vi "Periodic Tasks.vi"(8 "error in (no error)":errorcluster) -> ()   [LabVIEW 2016]
doc: "This VI runs in parallel to other tasks. It can contain as many user-defined periodic loops as you need. These can carry out PID or other sorts of timed response."
uses:
  Extra/TypeDefs/GatePos_Type.ctl
  Extra/TypeDefs/RobotParameters.ctl
  Extra/TypeDefs/GateParameters_Type.ctl
  ArgosLib/Miscellaneous/TypeDefs/MotorLimitPositions_Type.ctl
  Extra/TypeDefs/RailParameters_Type.ctl
  ArgosLib/Sensors/Ultrasonic/TypeDefs/UltrasonicParameters_Type.ctl
  Extra/TypeDefs/DB/dbParams_Type.ctl
  Extra/TypeDefs/AutoMode_Type.ctl
  ArgosLib/Drive/MotorControl/TypeDefs/RobotDriveMotorSelectorEnum.ctl
  Extra/TypeDefs/GearCollectState_Type.ctl
  Extra/TypeDefs/DB/dbButtonDisplayNames_Type.ctl
  Extra/TypeDefs/DB/dbStringDisplayNames_Type.ctl
  <vilib>/Rock Robotics/WPI/DriverStation/WPI_DriverStationRobotMode2.ctl
  Extra/TypeDefs/DB/dbSliderDisplayNames_Type.ctl
  <vilib>/Rock Robotics/WPI/ThirdParty/CanMotor/TalonSRX/WPI_CANTalonSRX_BrakeOverride.ctl
  Extra/Global_Var-RefNum/Global_Var_Drive.vi
  <vilib>/Rock Robotics/Network Tables/NT Write String.vi
  <vilib>/Rock Robotics/Network Tables/NT Read Boolean.vi
  <vilib>/Rock Robotics/Network Tables/NT Write Number.vi
  <vilib>/Rock Robotics/Network Tables/NT Write Boolean.vi
  Extra/Global_Var-RefNum/Global_Var_Other.vi
  <vilib>/Rock Robotics/Network Tables/NT Read String.vi
  Extra/Global_Var-RefNum/GlobalVar_LED.vi
  <vilib>/Rock Robotics/Network Tables/NT Read Number.vi
  ArgosLib/Miscellaneous/Arbitor/ArbitorSpecializations/Arbitor_Int.vi
  ArgosLib/Miscellaneous/Arbitor/ArbitorSpecializations/Arbitor_Float.vi
  ArgosLib/Miscellaneous/Arbitor/ArbitorSpecializations/Arbitor_Bool.vi
  ArgosLib/ArgosLib.lvlib
  Extra/Sensors/ADI MXP IMU/ADIS16448_IMU.lvlib
  Extra/Sensors/PixyCam/PixyCam_LabVIEW.lvlib
panel:
  in  "Continue_Forward_Distance":dbl=-15.0
  in  "BrakeMode?":bool
  in  "Turning_Angle":dbl=30.0
  in  "AutoMode":T1=enum."GearMiddle"
  in  "Reverse_Drive_Distance":dbl=-50.0 format="%#_13g"
  in  "Reverse_Drive_Speed":dbl=0.6 format="%#_13g"
  in  "Start_Auto?":bool
  in  "Robot Parameters":enum32{"Competition", "Practice"}(tab)
  in  "CompetitionRobotParameters":T2={"GateParameters"={"Scale Positions"={"Forward_StartScale"=1575.0, "Reverse_StartScale"=1440.0, "Forward_Limit"=1575.0, "Reverse_Limit"=1440.0}, "Catch_Pos"=1500.0, "Clamp_Pos"=1445.0, "Open_Pos"=1669.0, "Timeout (ms)"=750, "Invert?"=TRUE, "Scale_Factor"=0.01, "Acceptable_Range"=5.0}, "Rail Parameters"={"Scale Positions"={"Forward_StartScale"=15.4, "Reverse_StartScale"=8.7, "Forward_Limit"=21.4, "Reverse_Limit"=2.7}, "Motor_Limit"=0.6, "Invert?"=FALSE, "PID gains"={"proportional gain (Kc)"=0.2, "integral time (Ti, min)"=0.0, "derivative time (Td, min)"=0.0}, "Timeout (ms)"=2000, "CatchPosition"=6.5}, "Invert_Intake"=TRUE, "UltrasonicParameters"={"MedianFilterSamples"=8, "LowPassFilterPercent"=0.5, "RailOffset (in)"=4.0, "MaxRange (in)"=24.7}, "Feeder_Invert"=FALSE, "Drive PID Gains"={"proportional gain (Kc)"=0.04, "integral time (Ti, min)"=0.025, "derivative time (Td, min)"=1e-05}, "DriveSpeed_Invert"=TRUE, "DriveEncoder_Invert"=FALSE, "DefaultDBParams"={"MiddleAutoDist (in)"=-60.0, "SideAutoDist (in)"=-45.0, "AutoSpeed"=0.6, "RailCenterOffset (in)"=0.0, "RedAllianceRPM"=3550.0, "BlueAllianceRPM"=3400.0, "BaselineRPM"=3000.0}} {"Rail Parameters"."PID gains"."derivative time (Td, min)" format="%.3f"; "Rail Parameters"."PID gains"."integral time (Ti, min)" format="%.3f"; "Rail Parameters"."PID gains"."proportional gain (Kc)" format="%.3f"}
  in  "PracticeRobotParameters":T2={"GateParameters"={"Scale Positions"={"Forward_StartScale"=1700.0, "Reverse_StartScale"=1560.0, "Forward_Limit"=1700.0, "Reverse_Limit"=1560.0}, "Catch_Pos"=1620.0, "Clamp_Pos"=1585.0, "Open_Pos"=1680.0, "Timeout (ms)"=750, "Invert?"=TRUE, "Scale_Factor"=0.012, "Acceptable_Range"=5.0}, "Rail Parameters"={"Scale Positions"={"Forward_StartScale"=17.25, "Reverse_StartScale"=12.35, "Forward_Limit"=23.25, "Reverse_Limit"=6.35}, "Motor_Limit"=0.6, "Invert?"=FALSE, "PID gains"={"proportional gain (Kc)"=0.2, "integral time (Ti, min)"=0.0, "derivative time (Td, min)"=0.0}, "Timeout (ms)"=2000, "CatchPosition"=6.5}, "Invert_Intake"=FALSE, "UltrasonicParameters"={"MedianFilterSamples"=8, "LowPassFilterPercent"=0.5, "RailOffset (in)"=4.0, "MaxRange (in)"=27.0}, "Feeder_Invert"=FALSE, "Drive PID Gains"={"proportional gain (Kc)"=0.04, "integral time (Ti, min)"=0.025, "derivative time (Td, min)"=1e-05}, "DriveSpeed_Invert"=FALSE, "DriveEncoder_Invert"=TRUE, "DefaultDBParams"={"MiddleAutoDist (in)"=-60.0, "SideAutoDist (in)"=-45.0, "AutoSpeed"=0.6, "RailCenterOffset (in)"=0.0, "RedAllianceRPM"=3550.0, "BlueAllianceRPM"=3400.0, "BaselineRPM"=3000.0}} {"Rail Parameters"."PID gains"."derivative time (Td, min)" format="%.3f"; "Rail Parameters"."PID gains"."integral time (Ti, min)" format="%.3f"; "Rail Parameters"."PID gains"."proportional gain (Kc)" format="%.3f"}
  out "Ultrasonic":T8(graph)={"UltrasonicRange (in)"=1.824963579811325, "MedianOnly_UltrasonicRange (in)"=1.4520408163265301, "Unfiltered_UltrasonicRange (in)"=1.4513605442176853}
  in  "Manual_Track_Position":bool
  in  "Gear_Beam_Break_Sensor_Triggered":bool=TRUE
  in  "Reset_Encoder?":bool
  out "Dist_Travelled (In)":dbl
  out "Encoder Position":dbl
  out "Gear_Orientation_Bb_True?":bool
  in  "Manual_Gate_Control":T9
  out "Distance":dbl=-3.5761161830654182
  in  "GearRailWantedPosition":dbl(slide)=25.0 scale=5.0..25.0
  in  "ResetGearCollect":bool
  in  "ResetGearPlacer":bool
  in  "StartGearPlace":bool=TRUE
  in  "Place":bool=TRUE
  in  "Collect":bool=TRUE
  in  "Manual":bool
  in  "StartGearCollect":bool=TRUE
  out "GateReached":bool=TRUE
  out "IMU Angles Out":T10={"X Angle"=107.18836227857514, "Y Angle"=-158.5508446973779, "Z Angle"=83.6587271935076}
  # "Previous Values\nFwd_StartScale=1700\nReverse_StartScale=1560\nFwd_Limit=1700\nReverse_Limit=1560\nCatch=1604\nClamp=1570\nOpen=1669\nTimeout=750"
  # "1/24/17 (2014 Chassis)\nKc=0.015\nTi=5\nTd=0.0005\nTurns slowly, but well"
  # "2014 Chassis\nKc=0.09\nTi=0.9\nTd=0.001\nNot good for turning"
  # "2/12/17 (2017 Chassis)\nKc= 0.04\nTi=.025\nTd=1E-5\ndrives straight"
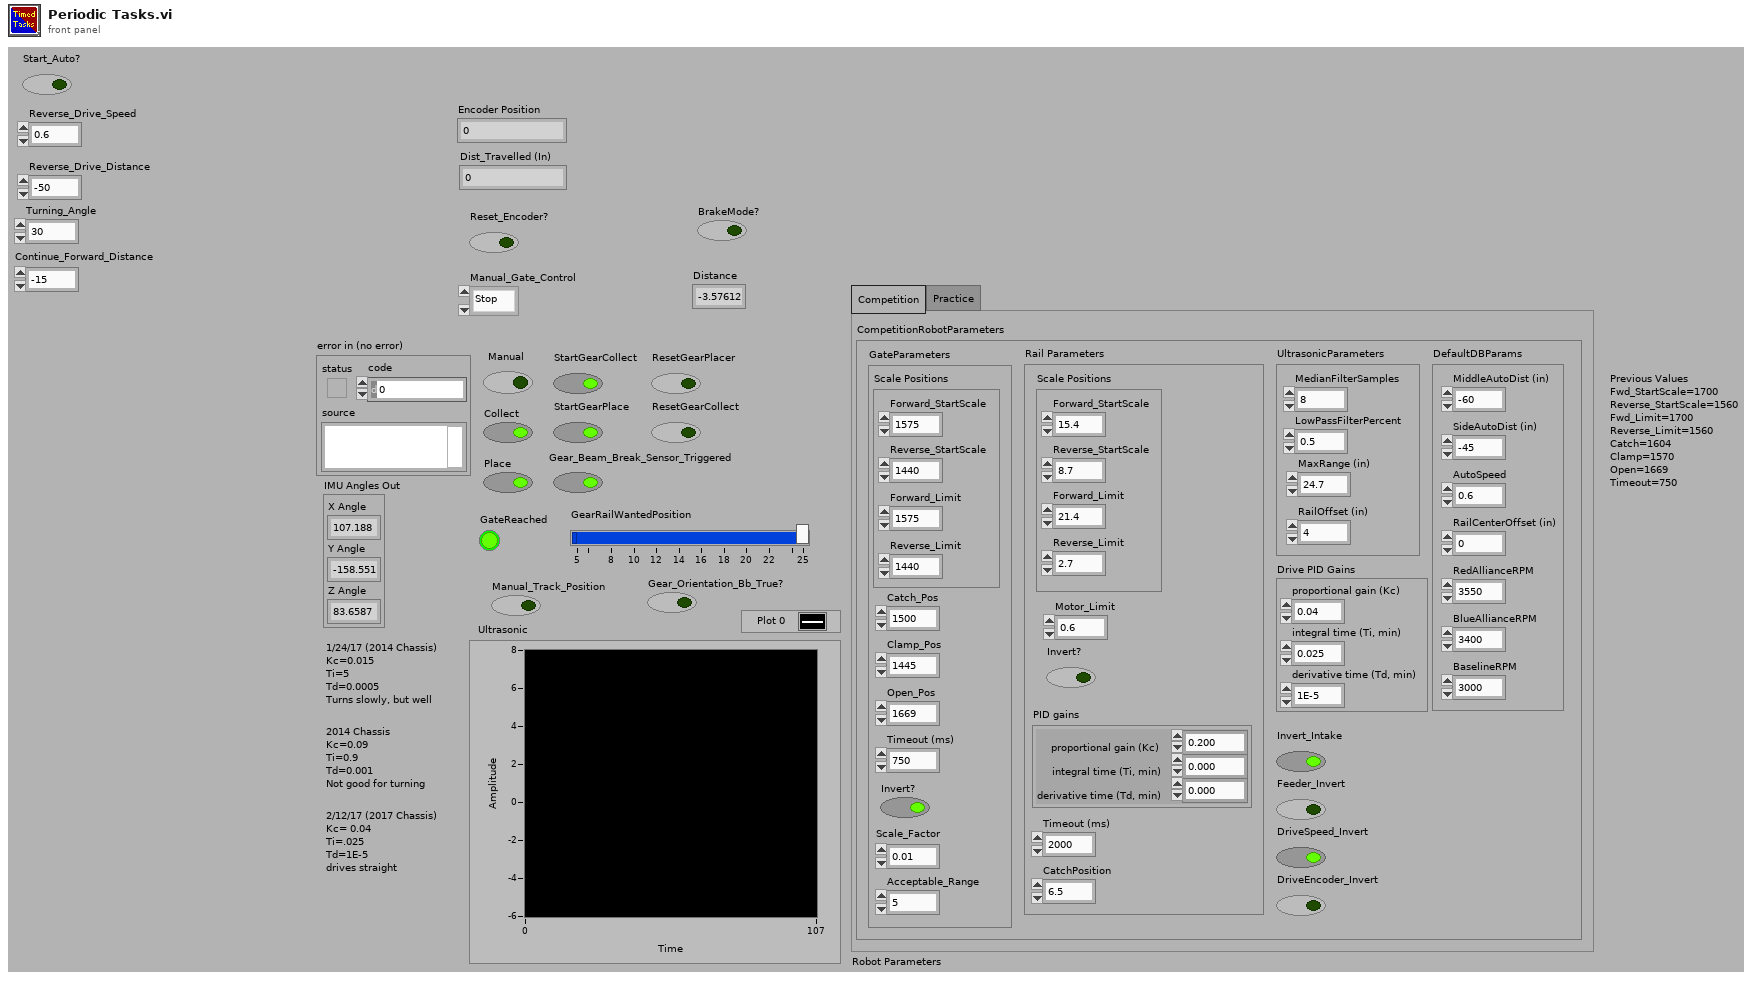
[diagram p1: front panel]
types:
  T1 = typedef "AutoMode_Type.ctl" = enum16{"GearRight", "GearMiddle", "GearLeft", "Shoot&GearMiddle", "BaselineOnly", "Shoot&Baseline"}
  T2 = typedef "RobotParameters.ctl" = cluster{"GateParameters":T3, "Rail Parameters":T5, "Invert_Intake":bool, "UltrasonicParameters":T6, "Feeder_Invert":bool, "Drive PID Gains":cluster{"proportional gain (Kc)":dbl, "integral time (Ti, min)":dbl, "derivative time (Td, min)":dbl}, "DriveSpeed_Invert":bool, "DriveEncoder_Invert":bool, "DefaultDBParams":T7}
  T3 = typedef "GateParameters_Type.ctl" = cluster{"Scale Positions":T4, "Catch_Pos":dbl, "Clamp_Pos":dbl, "Open_Pos":dbl, "Timeout (ms)":i32, "Invert?":bool, "Scale_Factor":dbl, "Acceptable_Range":dbl}
  T4 = typedef "MotorLimitPositions_Type.ctl" = cluster{"Forward_StartScale":dbl, "Reverse_StartScale":dbl, "Forward_Limit":dbl, "Reverse_Limit":dbl}
  T5 = typedef "RailParameters_Type.ctl" = cluster{"Scale Positions":T4, "Motor_Limit":dbl, "Invert?":bool, "PID gains":cluster{"proportional gain (Kc)":dbl, "integral time (Ti, min)":dbl, "derivative time (Td, min)":dbl}, "Timeout (ms)":u32, "CatchPosition":dbl}
  T6 = typedef "ArgosLib.lvlib/UltrasonicParameters_Type.ctl" = cluster{"MedianFilterSamples":u16, "LowPassFilterPercent":dbl, "RailOffset (in)":dbl, "MaxRange (in)":dbl}
  T7 = typedef "dbParams_Type.ctl" = cluster{"MiddleAutoDist (in)":dbl, "SideAutoDist (in)":dbl, "AutoSpeed":dbl, "RailCenterOffset (in)":dbl, "RedAllianceRPM":dbl, "BlueAllianceRPM":dbl, "BaselineRPM":dbl}
  T8 = cluster{"UltrasonicRange (in)":dbl, "MedianOnly_UltrasonicRange (in)":dbl, "Unfiltered_UltrasonicRange (in)":dbl}
  T9 = typedef "GatePos_Type.ctl" = enum16{"Stop", "Catch", "Clamp", "Open"}
  T10 = cluster{"X Angle":dbl, "Y Angle":dbl, "Z Angle":dbl}
  T11 = typedef "WPI_RobotDriveDevRef.ctl" = cluster{"DevStatus":errorcluster, "Motors[]":T12[], "Square Inputs":bool, "Max Output":dbl}
  T12 = typedef "WPI_MotorControlDeviceRef.ctl" = cluster{"DeviceStatus":errorcluster, "Type":T13, "PWM":cluster{"PWM Channel":T14, "DeadBand":T15}, "CAN":cluster{"Device Number":u8, "SetOutput VI Ref":variant, "GetOutput VI Ref":variant, "Enable VI Ref":variant, "Disable VI Ref":variant, "Data":variant}, "Invert":bool}
  T13 = typedef "WPI_MotorControlType.ctl" = enum16{"PWM", "CAN"}
  T14 = typedef "FPGA_DIOPWMChannel.ctl" = enum8{"PWM 0", "PWM 1", "PWM 2", "PWM 3", "PWM 4", "PWM 5", "PWM 6", "PWM 7", "PWM 8", "PWM 9", "PWM MXP 0", "PWM MXP 1", "PWM MXP 2", "PWM MXP 3", "PWM MXP 4", "PWM MXP 5", "PWM MXP 6", "PWM MXP 7", "PWM MXP 8", "PWM MXP 9", "Invalid"}
  T15 = typedef "WPI_PWMDeadband.ctl" = cluster{"Name":string, "maxPositivePwm":i32, "minPositivePwm":i32, "centerPwm":i32, "maxNegativePwm":i32, "minNegativePwm":i32, "angularRange":u16}
  T16 = typedef "PixyCam_LabVIEW.lvlib/PixyCam_DevRef.ctl" = cluster{"PixyCamDevRef_SPI":T17, "Communication Mode":T20, "Error":errorcluster}
  T17 = typedef "PixyCam_LabVIEW.lvlib/PixyCam_SPI_DevRef.ctl" = cluster{"SPIDevRef":T18, "Output Queue":refnum<queue>}
  T18 = typedef "WPI_SPIDevRef.ctl" = cluster{"DevStatus":errorcluster, "Handle":i32, "SPI Bus":T19}
  T19 = typedef "spi_bus.ctl" = enum16{"SPI On-Board, CS0", "SPI On-Board, CS1", "SPI On-Board, CS2", "SPI On-Board, CS3", "SPI MXP", "Invalid"}
  T20 = typedef "PixyCam_LabVIEW.lvlib/PixyCam_CommMode.ctl" = enum16{"SPI", "I2C", "UART", "Analog", "Digital"}
  T21 = typedef "ADIS16448_IMU.lvlib/ADI_IMU_ADIS16448_InterruptDevRef.ctl" = cluster{"ADI IMU DevRef":T22, "InterruptRef":T23}
  T22 = typedef "ADIS16448_IMU.lvlib/ADI_IMU_ADIS16448_IMUDevRef.ctl" = cluster{"DevStatus":errorcluster, "Handle":i32, "SPI Bus":T19, "Device Found":bool, "Device Ready":bool, "Yaw Axis":enum16{"X", "Y", "Z"}, "AHRS Algorithm":enum16{"Complementary", "Madgwick"}, "Serial":u16, "Lot ID 2":u16, "Lot ID 1":u16, "Product ID":u16}
  T23 = typedef "WPI_InterruptRef.ctl" = cluster{"DevStatus":errorcluster, "InterruptIndex":T24}
  T24 = typedef "FPGA_InterruptIndex.ctl" = enum8{"0", "1", "2", "3", "4", "5", "6", "7", "Invalid"}
  T25 = typedef "WPI_AnalogChannelDevRef.ctl" = cluster{"DevStatus":errorcluster, "Analog Channel":T26}
  T26 = typedef "FPGA_AIChannel.ctl" = enum8{"AI 0", "AI 1", "AI 2", "AI 3", "AI MXP 0", "AI MXP 1", "AI MXP 2", "AI MXP 3", "Invalid"}
  T27 = typedef "WPI_SonarMB1010DigitalDeviceRef.ctl" = cluster{"CounterDevRef":T28, "Scaling factor (s/in)":dbl}
  T28 = typedef "WPI_CounterDevRef.ctl" = cluster{"DevStatus":errorcluster, "CntIndex":T29}
  T29 = typedef "FPGA_CounterCtrSystemIndex.ctl" = enum8{"Ctr 0", "Ctr 1", "Ctr 2", "Ctr 3", "Ctr 4", "Ctr 5", "Ctr 6", "Ctr 7", "Invalid"}
  T30 = typedef "WPI_EncoderDevRef.ctl" = cluster{"DevStatus":errorcluster, "EncoderIndex":T31, "CounterIndex":T29, "DistancePerCount":dbl, "Decoding Type":T32}
  T31 = typedef "FPGA_EncoderIdx.ctl" = enum8{"Enc 0", "Enc 1", "Enc 2", "Enc 3", "Enc 4", "Enc 5", "Enc 6", "Enc 7", "Invalid"}
  T32 = typedef "WPI_EncoderType.ctl" = enum16{"1x", "2x", "4x"}
  T33 = typedef "WPI_DigitalInputDevRef.ctl" = cluster{"DevStatus":errorcluster, "DIO Channel":T34}
  T34 = typedef "FPGA_DIOChannel.ctl" = enum8{"DIO 0", "DIO 1", "DIO 2", "DIO 3", "DIO 4", "DIO 5", "DIO 6", "DIO 7", "DIO 8", "DIO 9", "DIO MXP 0", "DIO MXP 1", "DIO MXP 2", "DIO MXP 3", "DIO MXP 4", "DIO MXP 5", "DIO MXP 6", "DIO MXP 7", "DIO MXP 8", "DIO MXP 9", "DIO MXP 10", "DIO MXP 11", "DIO MXP 12", "DIO MXP 13", "DIO MXP 14", "DIO MXP 15", "SPI Port CS1", "SPI Port CS2", "SPI Port CS3", "SPI Port MISO", "SPI Port MOSI", "Invalid"}
  T35 = typedef "WPI_CompressorDevRef.ctl" = cluster{"DevStatus":errorcluster, "Pneumatics Control Module":u8}
  T36 = typedef "WPI_SolenoidDevRef.ctl" = cluster{"DevStatus":errorcluster, "Pneumatics Control Module":u8, "Forward Solenoid Channel":T37, "Reverse Solenoid Channel":T37}
  T37 = typedef "WPI_SolenoidChannel.ctl" = enum8{"Solenoid 0", "Solenoid 1", "Solenoid 2", "Solenoid 3", "Solenoid 4", "Solenoid 5", "Solenoid 6", "Solenoid 7", "Invalid"}
  T38 = cluster{"Motors":cluster{"Drive_Motor":cluster{"RobotDriveDevRef":T11, "error out":errorcluster}, "Left_Shooter":cluster{"MotorControlDevRef":T12, "error out":errorcluster}, "Shooter_Feeder_Motor":cluster{"MotorControlDevRef":T12, "error out":errorcluster}, "Intake_Motor_1":cluster{"MotorControlDevRef":T12, "error out":errorcluster}, "Gear_Gate_Motor":cluster{"MotorControlDevRef":T12, "error out":errorcluster}, "Climber_Motor":cluster{"MotorControlDevRef":T12, "error out":errorcluster}, "Left_Turret":cluster{"MotorControlDevRef":T12, "error out":errorcluster}, "Right_Shooter":cluster{"MotorControlDevRef":T12, "error out":errorcluster}, "Gear_Rail_Motor":cluster{"MotorControlDevRef":T12, "error out":errorcluster}}, "Sensors":cluster{"PixyCam":cluster{"PixyCamDevRef Out":T16, "error out":errorcluster}, "IMU":cluster{"ADI IMU Interrupt DevRef":T21, "error out":errorcluster}, "Pots":cluster{"Gear_Gate_Pot":cluster{"AIDeviceRef":T25, "error out":errorcluster}, "Gear_Rail_Pot":cluster{"AIDeviceRef":T25, "error out":errorcluster}, "Turret_Pot":cluster{"AIDeviceRef":T25, "error out":errorcluster}}, "Ultrasonics":cluster{"Gear_Peg_Ultrasonic":cluster{"SonarMB1010DigitalDevRef":T27, "error out":errorcluster}}, "Encoders":cluster{"Drive_Encoder":cluster{"EncoderDevRef":T30, "error out":errorcluster}, "Shooter_Encoder":cluster{"EncoderDevRef":T30, "error out":errorcluster}}, "DIOs":cluster{"Gear_Beambreak":cluster{"DigitalInputDevRef":T33, "error out":errorcluster}, "Ball_Beambreak":cluster{"DigitalInputDevRef":T33, "error out":errorcluster}, "Gear_Orientation_Beambreak":cluster{"DigitalInputDevRef":T33, "error out":errorcluster}}}, "Pneumatics":cluster{"Compressor":cluster{"CompressorDevRef":T35, "error out":errorcluster}, "Gear_Pusher":cluster{"SolenoidDevRef":T36, "error out":errorcluster}, "Shifters":cluster{"SolenoidDevRef":T36, "error out":errorcluster}, "Gear_Chute":cluster{"SolenoidDevRef":T36, "error out":errorcluster}}}
  T39 = typedef "dbStringDisplayNames_Type.ctl" = enum16{"RedAllianceRPM", "Drive P", "Drive I", "Drive D", "String 4", "BlueAllianceRPM", "BaselineRPM", "String 7", "String 8", "String 9"}
  T40 = typedef "dbButtonDisplayNames_Type.ctl" = enum16{"ResetValues", "CATCH", "CATCH ", "CATCH  "}
  T41 = typedef "GearCollectState_Type.ctl" = enum16{"Store Gear", "Wait For Gear", "Idle"}
  T42 = typedef "ArgosLib.lvlib/RobotDriveMotorSelectorEnum.ctl" = enum16{"Left Motor 1", "Right Motor 1", "Left Motor 2", "Right Motor 2", "Left Motor 3", "Right Motor 3"}
  T43 = typedef "dbSliderDisplayNames_Type.ctl" = enum16{"MiddleAutoDist (in)", "SideAutoDist (in)", "AutoSpeed", "RailCenterOffset (in)"}
  T44 = typedef "WPI_CANTalonSRX_GlobalStatus.ctl" = cluster{"Applied Throttle":dbl, "Module Enabled":bool, "CAN Error":errorcluster, "Closed Loop Error":dbl, "Forward Limit Switch Closed":bool, "Reverse Limit Switch Closed":bool, "Sensor Position":dbl, "Sensor Velocity":dbl, "Current":dbl, "Sticky Fault - Over Temp":bool, "Sticky Fault - Under Voltage":bool, "Sticky Fault - Forward Limit":bool, "Sticky Fault - Reverse Limit":bool, "Sticky Fault - Forward Soft Limit":bool, "Sticky Fault - Reverse Soft Limit":bool, "Brake is Enabled":bool, "Encoder Position":dbl, "Encoder Velocity":dbl, "Encoder Index Count":dbl, "Encoder A Pin State":bool, "Encoder B Pin State":bool, "Encoder Index Pin State":bool, "Analog In":dbl, "Analog In Velocity":dbl, "Temperature (C)":dbl, "Battery Voltage":dbl, "Control 5 Is Supported":bool, "Current Profile Slot Select":dbl, "Pos Div 8":bool, "Vel Div 4":bool, "Pulse Width Position":i32, "Pulse Width Velocity":i32, "Pulse Width Rise To Rise (us)":i32, "Pulse Width Rise To Fall (us)":i32, "Mot Prof Active Is Under Run":bool, "Mot Prof Active Has Under Run":bool, "Mot Prof Active Is Last":bool, "Mot Prof Active Velocity Only":bool, "Mot Prof Active Is Valid":bool, "Mot Prof Buffer Is Full":bool, "Mot Prof Active Profile Slot Select":i32, "Mot Prof NextID":i32, "Mot Prof Count":i32, "Mot Prof Active Velocity":dbl, "Mot Prof Active Position":dbl, "Mot Prof Output Enable":i32}
  T45 = cluster{"proportional gain (Kc)":dbl, "integral time (Ti, min)":dbl, "derivative time (Td, min)":dbl}
  T46 = typedef "WPI_DriverStationRobotMode2.ctl" = enum16{"Autonomous Disabled", "Autonomous Enabled", "Teleop Disabled", "Teleop Enabled", "Disconnected", "Finish", "Test Disabled", "Test Enabled", "Emergency Stopped"}
  T47 = typedef "WPI_CANTalonSRX_BrakeOverride.ctl" = enum8{"No Override", "Override to Coast", "Override to Brake"}
  T48 = cluster{"Joystick_1":cluster{"Joystick_Unassigned":dbl, "Joystick_F/B":dbl, "Joystick_L/R_Turn":dbl, "Joysick_Unassigned":dbl, "Joystick_Unassigned":dbl, "Joystick_Gearpusher":bool, "Joystick_Climb":bool, "Joystick_Intake":bool, "Joystick_Place_Gear":bool, "Joystick_DriveStraight":bool, "Joysick_Shoot":bool, "Joystick_Shift":bool, "Joystick_Aim":bool, "Joysick_Lightshow":bool}, "Joystick_2":cluster{"Joystick_GearRail_R/L":dbl, "Joystick_Climb_UpDown":dbl, "Joystick_Turret_L/R":dbl, "Joystick_Unassigned":dbl, "Joystick_BotFeed_F":bool, "Joystick_BotFeed_B":bool, "Joystick_GateOpen":bool, "Joystick_GateClose":bool, "Joystick_GateClamp":bool, "Joystick_Intake_B":bool, "Joystick_Feed_F":bool, "Joysitick_Feed_B":bool, "Joystick_GearChute":bool, "Joystick_Unassigned":dbl, "Joystick_ResetCatch":bool}}
  T49 = typedef "TurretAimState_Type.ctl" = enum16{"Idle", "SearchLeft", "SearchRight", "FindNewTarget", "TargetAcquired"}
  T50 = typedef "WPI_DriverStationAllianceInfo.ctl" = enum16{"Red", "Blue", "Invalid"}
  T51 = typedef "GearPlaceState_Type.ctl" = enum16{"Idle", "Wait for Peg", "Allign To Lift", "Arm Gear", "Place Gear", "Return to Ready", "Disarm Gear"}
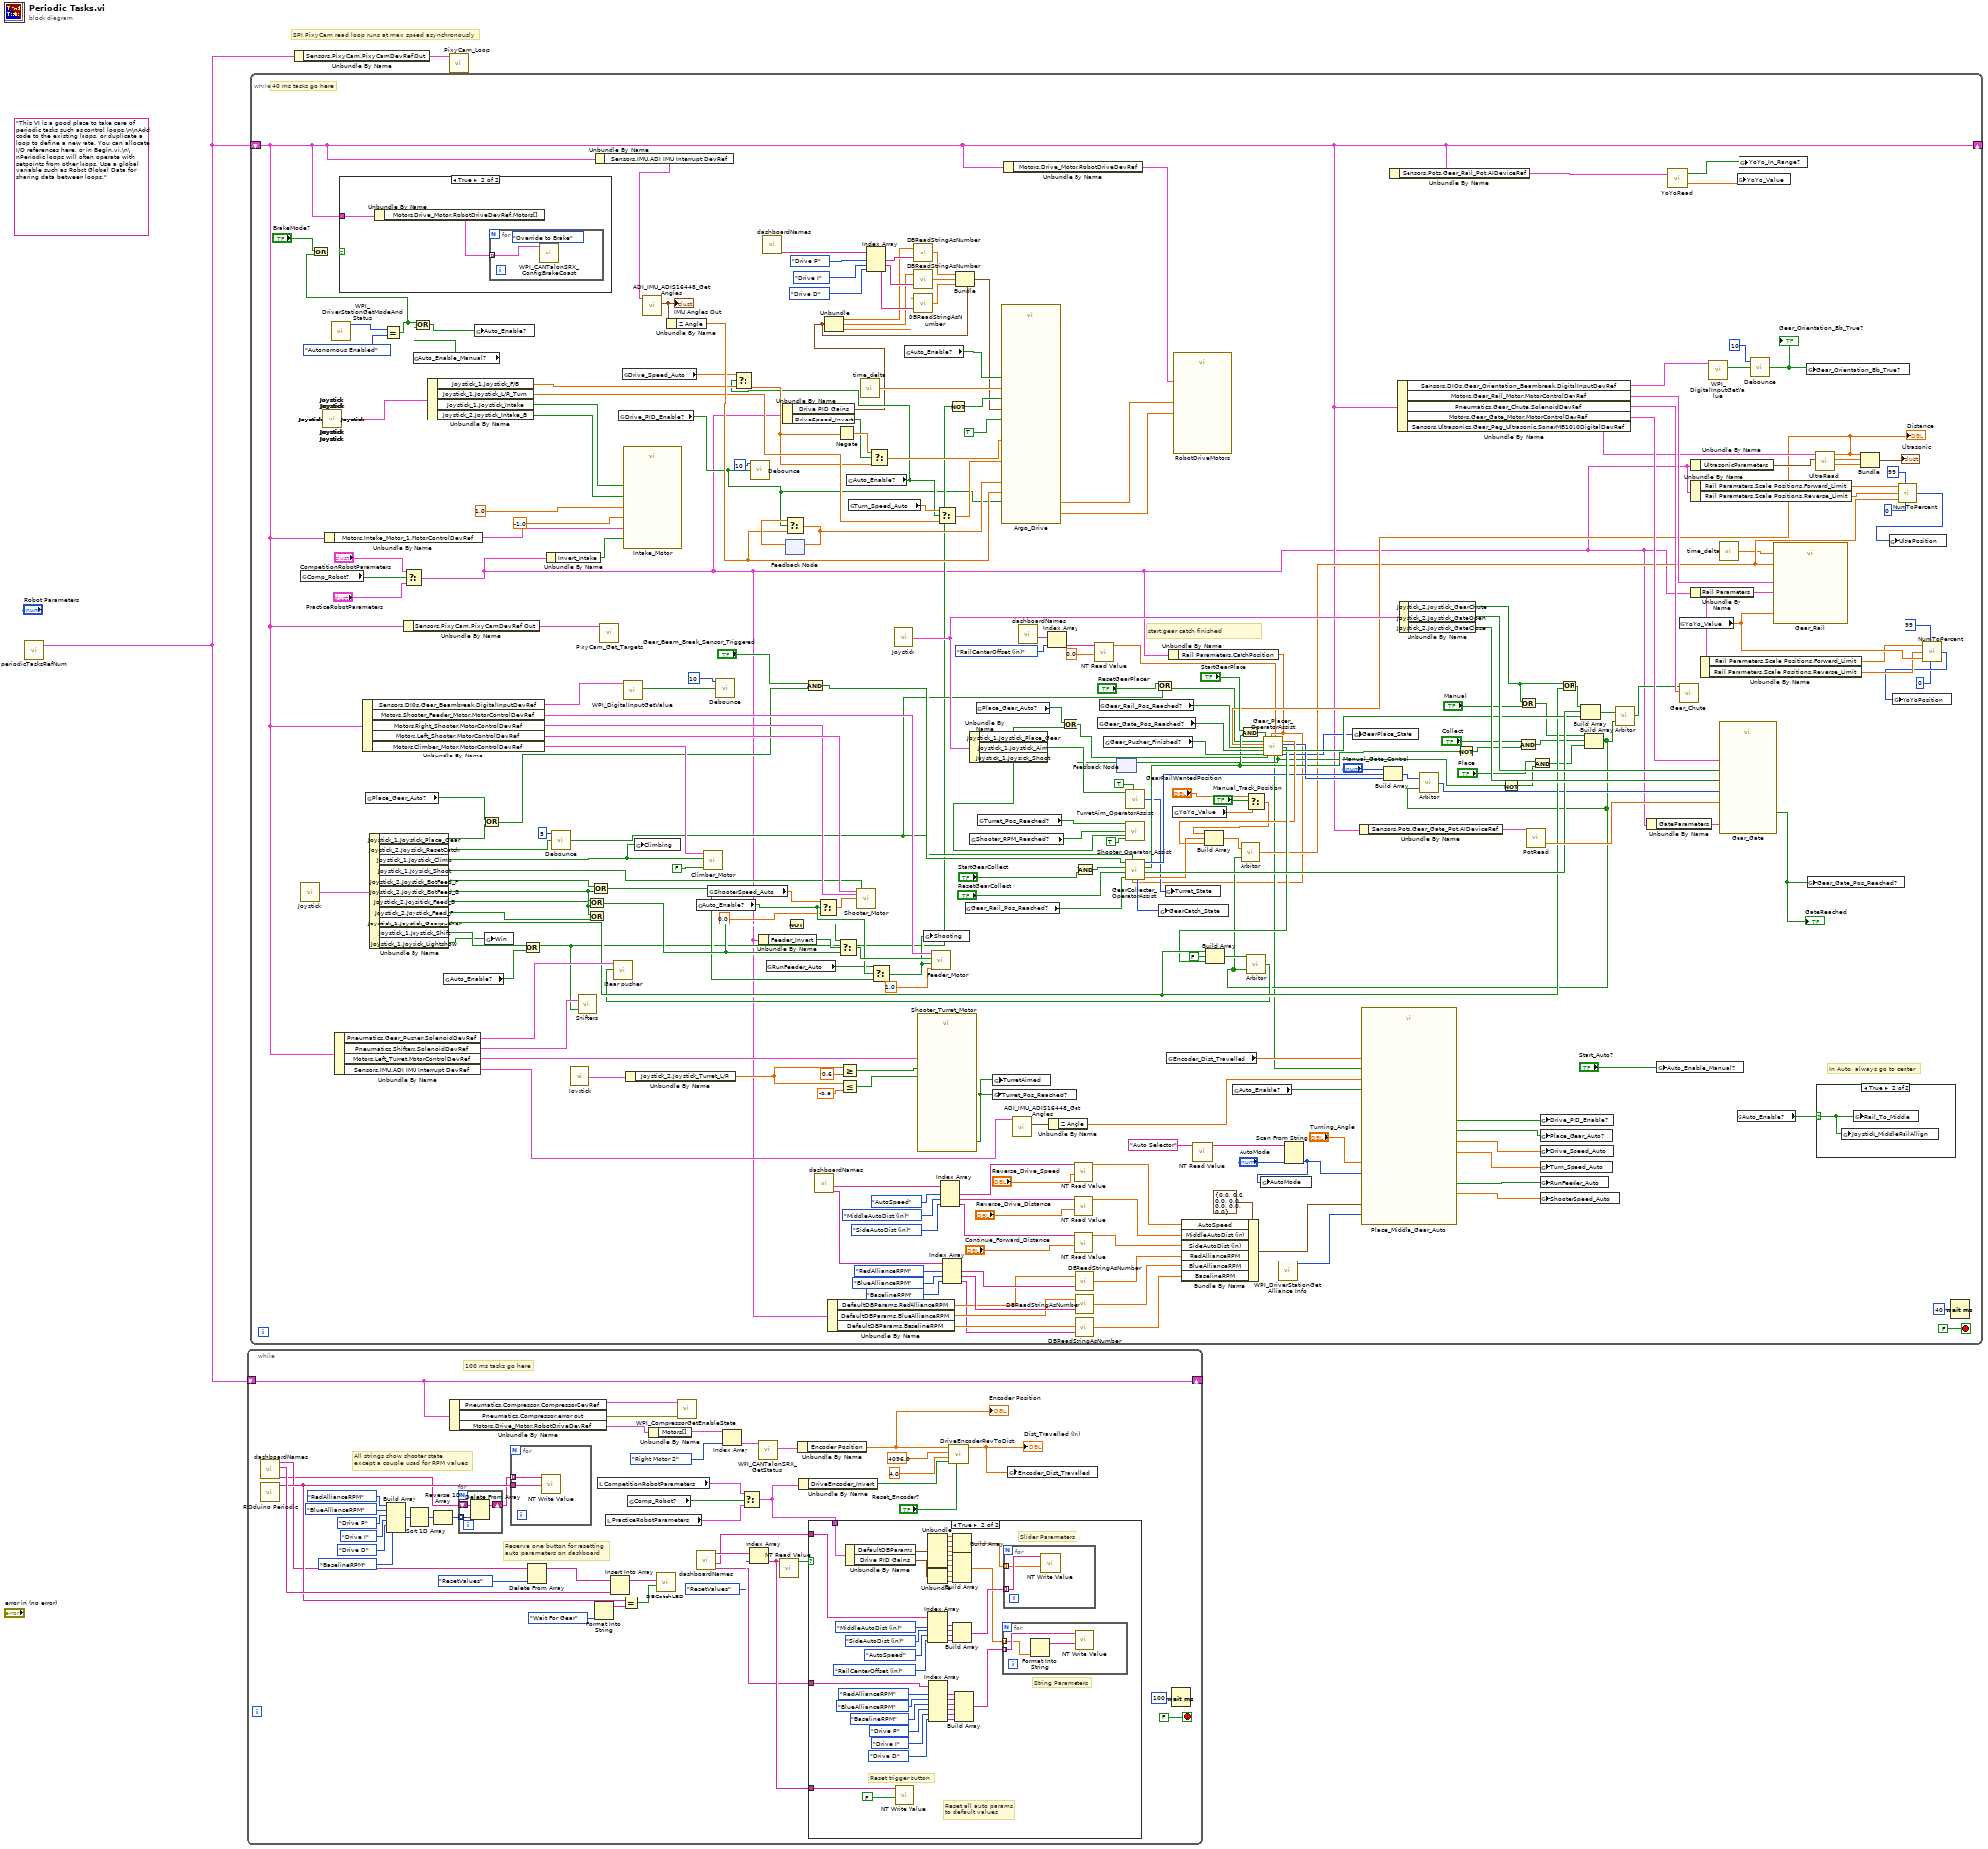
[diagram p0: block diagram]
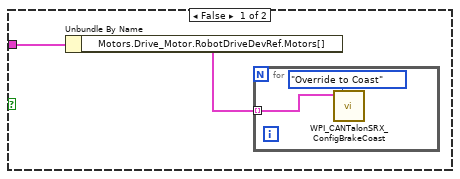
[diagram p4: hidden frame]
diagram:
  (unwired) "This VI is a good place to take care of periodic tasks such as control loops.\n\nAdd code to the existing loops, or duplicate a loop to define a new rate. You can allocate I/O references here, or in Begin.vi.\n\nPeriodic loops will often operate with setpoints from other loops. Use a global variable such as Robot Global Data for sharing data between loops."
  # "SPI PixyCam read loop runs at max speed asynchronously"
  n1 = call "periodicTasksRefNum.vi"() -> ("Refnums"=w2:T38)  [unwired: 3 in]
  n2 = while {
    shift-right: [w46] -> _
    shift-left: w2 -> [w46]
    stop <- FALSE stop-if-true
    # "All strings show shooter state\nexcept a couple used for RPM values"
    # "Reserve one button for resetting\nauto parameters on dashboard"
    # "100 ms tasks go here"
    n3 = call "dashboardNames.vi"() -> ("String Names"=w8:string[], "LED Names"=w29:string[], "Button Names"=w23:string[])  [unwired: 8 in, 1 out]
    n4 = call "RIOduino Periodic.vi"() -> ("GearMode"=w26:string)  [unwired: 11 in]
    n5 = Build Array(dbStringDisplayNames_Type."RedAllianceRPM" ("DBSliderDispNames"), dbStringDisplayNames_Type."BlueAllianceRPM" ("DBSliderDispNames"), dbStringDisplayNames_Type."Drive P" ("DBSliderDispNames"), dbStringDisplayNames_Type."Drive I" ("DBSliderDispNames"), dbStringDisplayNames_Type."Drive D" ("DBSliderDispNames"), dbStringDisplayNames_Type."BaselineRPM" ("DBSliderDispNames")) -> (w11:T39[])
    n6 = Sort 1D Array(array=w11) -> (sorted array=w10:T39[])
    n7 = Reverse 1D Array(array=w10) -> (reversed array=w9:T39[])
    n8 = Unbundle By Name(w46) -> ("Pneumatics.Compressor.CompressorDevRef"=w45:T35, "Pneumatics.Compressor.error out"=w44:errorcluster, "Motors.Drive_Motor.RobotDriveDevRef"=w43:T11)
    n9 = for {
      tunnel: w9 -> [w51] mode=indexing
      shift-right: [w49] -> w7
      shift-left: w8 -> [w50]
      n10 = Delete From Array(array=w50, index=w51) -> (array with subset deleted=w49:string[])  [unwired: 1 in, 1 out]
    }
    n11 = for {
      tunnel: w7 -> [w99] mode=indexing
      tunnel: w26 -> [w98]
      n12 = call-poly <vilib>:"NT Write Value.vi"("String"=w98, "Name"=w99) -> ()  [unwired: 9 in, 1 out]
    }
    n13 = Delete From Array(array=w23, index=dbButtonDisplayNames_Type."ResetValues" ("DBButtonDispNames")) -> (array with subset deleted=w21:string[])  [unwired: 1 in, 1 out]
    n14 = Format Into String(GearCollectState_Type."Wait For Gear" ("Current_State")) -> (resulting string=w27:string)  [unwired: 3 in, 1 out]
    n15 = local read "CompetitionRobotParameters"() -> (w33:T2)
    n16 = local read "PracticeRobotParameters"() -> (w32:T2)
    n17 = Insert Into Array(array=w21, new element=w29) -> (w24:string[])  [unwired: 1 in]
    n18 = Equal?(x=w26, y=w27) -> (x = y?=w25:bool)
    n19 = global read "Global_Var_Drive.vi" "Comp_Robot?"() -> (w31:bool)
    n20 = Unbundle By Name(w43) -> ("Motors[]"=w42:T12[])
    n21 = call "DBCatchLED.vi"("Catch"=w25, "DBNames"=w24) -> ()  [unwired: 10 in]
    n22 = call <vilib>:"WPI_CompressorGetEnableState.vi"("error in (no error)"=w44, "CompressorDevRef"=w45) -> ()  [unwired: 6 in, 4 out]
    n23 = call "dashboardNames.vi"() -> ("String Names"=w14:string[], "Slider Names"=w16:string[], "Button Names"=w20:string[])  [unwired: 8 in, 1 out]
    n24 = Index Array(array=w42, index=RobotDriveMotorSelectorEnum."Right Motor 2" ("Motor Selector Enum")) -> (element=w40:T12)
    n25 = Select(t=w33, s=w31, f=w32) -> (s? t:f=w15:T2)
    n26 = Index Array(array=w20, index=dbButtonDisplayNames_Type."ResetValues" ("DBButtonDispNames")) -> (element=w17:string)
    n27 = call <vilib>:"WPI_CANTalonSRX_GetStatus.vi"("CAN Talon SRX Ref"=w40) -> ("Talon SRX Status"=w39:T44)  [unwired: 8 in, 2 out]
    n28 = call-poly <vilib>:"NT Read Value.vi"("Name"=w17) -> ("Boolean"=w18:bool)  [unwired: 9 in, 1 out]
    n29 = Unbundle By Name(w39) -> ("Encoder Position"=w38:dbl)
    "Encoder Position" <- w38
    n30 = Unbundle By Name(w15) -> ("DriveEncoder_Invert"=w30:bool)
    n31 = case shown="True" w18 {
      tunnel: w17 -> [_ w92]
      tunnel: w16 -> [_ w90]
      tunnel: w15 -> [_ w85]
      tunnel: w14 -> [_ w73]
      frame False {
        # "Do nothing"
      }
      frame True {
        # "Slider Parameters"
        # "String Parameters"
        # "Reset all auto params\nto default values"
        # "Reset trigger button"
        n32 = Unbundle By Name(w85) -> ("DefaultDBParams"=w84:T7, "Drive PID Gains"=w63:T45)
        n33 = call-poly <vilib>:"NT Write Value.vi"("Boolean"=FALSE, "Name"=w92) -> ()  [unwired: 9 in, 1 out]
        n34 = Unbundle(w84) -> ("MiddleAutoDist (in)"=w83:dbl, "SideAutoDist (in)"=w82:dbl, "AutoSpeed"=w81:dbl, "RailCenterOffset (in)"=w80:dbl, "RedAllianceRPM"=w59:dbl, "BlueAllianceRPM"=w58:dbl, "BaselineRPM"=w57:dbl)
        n35 = Unbundle(w63) -> ("proportional gain (Kc)"=w62:dbl, "integral time (Ti, min)"=w61:dbl, "derivative time (Td, min)"=w60:dbl)
        n36 = Index Array(array=w90, index #1=dbSliderDisplayNames_Type."MiddleAutoDist (in)" ("DBSliderDispNames"), index #2=dbSliderDisplayNames_Type."SideAutoDist (in)" ("DBSliderDispNames"), index #3=dbSliderDisplayNames_Type."AutoSpeed" ("DBSliderDispNames"), index #4=dbSliderDisplayNames_Type."RailCenterOffset (in)" ("DBSliderDispNames")) -> (element #1=w79:string, element #2=w78:string, element #3=w77:string, element #4=w76:string)
        n37 = Index Array(array=w73, index #1=dbStringDisplayNames_Type."RedAllianceRPM" ("DBSliderDispNames"), index #2=dbStringDisplayNames_Type."BlueAllianceRPM" ("DBSliderDispNames"), index #3=dbStringDisplayNames_Type."BaselineRPM" ("DBSliderDispNames"), index #4=dbStringDisplayNames_Type."Drive P" ("DBSliderDispNames"), index #5=dbStringDisplayNames_Type."Drive I" ("DBSliderDispNames"), index #6=dbStringDisplayNames_Type."Drive D" ("DBSliderDispNames")) -> (element #1=w69:string, element #2=w68:string, element #3=w66:string, element #4=w65:string, element #5=w64:string, element #6=w56:string)
        n38 = Build Array(w83, w82, w81, w80) -> (w75:dbl[])
        n39 = Build Array(w59, w58, w57, w62, w61, w60) -> (w70:dbl[])
        n40 = Build Array(w79, w78, w77, w76) -> (w74:string[])
        n41 = Build Array(w69, w68, w66, w65, w64, w56) -> (w67:string[])
        n42 = for {
          tunnel: w70 -> [w93] mode=indexing
          tunnel: w67 -> [w95] mode=indexing
          n43 = Format Into String(w93) -> (resulting string=w94:string)  [unwired: 3 in, 1 out]
          n44 = call-poly <vilib>:"NT Write Value.vi"("String"=w94, "Name"=w95) -> ()  [unwired: 9 in, 1 out]
        }
        n45 = for {
          tunnel: w75 -> [w96] mode=indexing
          tunnel: w74 -> [w97] mode=indexing
          n46 = call-poly <vilib>:"NT Write Value.vi"("Numeric"=w96, "Name"=w97) -> ()  [unwired: 9 in, 1 out]
        }
      }
    }
    n47 = call "DriveEncoderRevToDist.vi"("Reset_Encoder?"="Reset_Encoder?", "Invert?"=w30, "Wheel_Diameter (In)"=4.0, "Counts_Per_Rev"=4096.0, "Encoder_Rev_Count"=w38) -> ("Dist_Travelled (In)"=w34:dbl)  [unwired: 6 in]
    "Dist_Travelled (In)" <- w34
    n48 = global write "Global_Var_Other.vi" "Encoder_Dist_Travelled"(w34) -> ()
    n49 = Wait (ms)(milliseconds to wait=u32 100) -> ()  [unwired: 1 out]
  }
  n50 = while {
    shift-right: [w157] -> _
    shift-left: w2 -> [w157]
    stop <- FALSE stop-if-true
    # "In Auto, always go to center"
    # "start:gear catch finished"
    # "40 ms tasks go here"
    n51 = call "Joystick.vi"() -> ("Joysticks"=w320:T48)  [unwired: 1 in]
    n52 = global read "Global_Var_Drive.vi" "Comp_Robot?"() -> (w241:bool)
    n53 = call "Joystick.vi"() -> ()  [unwired: 1 in, 1 out]
    n54 = call "Joystick.vi"() -> ()  [unwired: 1 in, 1 out]
    n55 = call "Joystick.vi"() -> ()  [unwired: 1 in, 1 out]
    n56 = call "Joystick.vi"() -> ()  [unwired: 1 in, 1 out]
    n57 = call "Joystick.vi"() -> ()  [unwired: 1 in, 1 out]
    n58 = call "Joystick.vi"() -> ()  [unwired: 1 in, 1 out]
    n59 = call "Joystick.vi"() -> ()  [unwired: 1 in, 1 out]
    n60 = call "Joystick.vi"() -> ()  [unwired: 1 in, 1 out]
    n61 = call "Joystick.vi"() -> ()  [unwired: 1 in, 1 out]
    n62 = call "Joystick.vi"() -> ()  [unwired: 1 in, 1 out]
    n63 = call "Joystick.vi"() -> ()  [unwired: 1 in, 1 out]
    n64 = call "Joystick.vi"() -> ()  [unwired: 1 in, 1 out]
    n65 = call "Joystick.vi"() -> ()  [unwired: 1 in, 1 out]
    n66 = call "Joystick.vi"() -> ()  [unwired: 1 in, 1 out]
    n67 = call "Joystick.vi"() -> ()  [unwired: 1 in, 1 out]
    n68 = call "Joystick.vi"() -> ()  [unwired: 1 in, 1 out]
    n69 = call "Joystick.vi"() -> ()  [unwired: 1 in, 1 out]
    n70 = call "Joystick.vi"() -> ()  [unwired: 1 in, 1 out]
    n71 = call "Joystick.vi"() -> ()  [unwired: 1 in, 1 out]
    n72 = call "Joystick.vi"() -> ()  [unwired: 1 in, 1 out]
    n73 = call "Joystick.vi"() -> ()  [unwired: 1 in, 1 out]
    n74 = call "Joystick.vi"() -> ("Joysticks"=w334:T48)  [unwired: 1 in]
    n75 = Unbundle By Name(w157) -> ("Motors.Intake_Motor_1.MotorControlDevRef"=w324:T12)
    n76 = call <vilib>:"WPI_DriverStationGetModeAndStatus.vi"() -> ("Robot Mode"=w218:T46)  [unwired: 10 in, 1 out]
    n77 = Unbundle By Name(w157) -> ("Pneumatics.Gear_Pusher.SolenoidDevRef"=w315:T36, "Pneumatics.Shifters.SolenoidDevRef"=w314:T36, "Motors.Left_Turret.MotorControlDevRef"=w313:T12, "Sensors.IMU.ADI IMU Interrupt DevRef"=w257:T21)
    n78 = Unbundle By Name(w157) -> ("Sensors.DIOs.Gear_Beambreak.DigitalInputDevRef"=w264:T33, "Motors.Shooter_Feeder_Motor.MotorControlDevRef"=w316:T12, "Motors.Right_Shooter.MotorControlDevRef"=w228:T12, "Motors.Left_Shooter.MotorControlDevRef"=w317:T12, "Motors.Climber_Motor.MotorControlDevRef"=w318:T12)
    n79 = global read "Global_Var_Other.vi" "Place_Gear_Auto?"() -> (w222:bool)
    n80 = Unbundle By Name(w320) -> ("Joystick_1.Joystick_Place_Gear"=w223:bool, "Joystick_2.Joystick_ResetCatch"=w179:bool, "Joystick_1.Joystick_Climb"=w208:bool, "Joystick_1.Joysick_Shoot"=w193:bool, "Joystick_2.Joystick_BotFeed_F"=w311:bool, "Joystick_2.Joystick_BotFeed_B"=w312:bool, "Joystick_2.Joysitick_Feed_B"=w335:bool, "Joystick_2.Joystick_Feed_F"=w336:bool, "Joystick_1.Joystick_Gearpusher"=w293:bool, "Joystick_1.Joystick_Shift"=w337:bool, "Joystick_1.Joysick_Lightshow"=w209:bool)
    n81 = Equal?(x=w218, y=WPI_DriverStationRobotMode2."Autonomous Enabled" ("Robot Mode")) -> (x = y?=w158:bool)
    n82 = Or(x="BrakeMode?", y=w158) -> (x .or. y?=w156:bool)
    n83 = case shown="True" w156 {
      tunnel: w157 -> [w361 w365]
      frame False {
        n84 = Unbundle By Name(w361) -> ("Motors.Drive_Motor.RobotDriveDevRef.Motors[]"=w360:T12[])
        n85 = for {
          tunnel: w360 -> [w363] mode=indexing
          n86 = call <vilib>:"WPI_CANTalonSRX_ConfigBrakeCoast.vi"("Brake / Coast Mode"=WPI_CANTalonSRX_BrakeOverride."Override to Coast", "CAN Talon SRX Ref"=w363) -> ()  [unwired: 8 in, 2 out]
        }
      }
      frame True {
        n87 = Unbundle By Name(w365) -> ("Motors.Drive_Motor.RobotDriveDevRef.Motors[]"=w364:T12[])
        n88 = for {
          tunnel: w364 -> [w367] mode=indexing
          n89 = call <vilib>:"WPI_CANTalonSRX_ConfigBrakeCoast.vi"("Brake / Coast Mode"=WPI_CANTalonSRX_BrakeOverride."Override to Brake", "CAN Talon SRX Ref"=w367) -> ()  [unwired: 8 in, 2 out]
        }
      }
    }
    n90 = Unbundle By Name(w157) -> ("Sensors.PixyCam.PixyCamDevRef Out"=w308:T16)
    n91 = Select(t="CompetitionRobotParameters", s=w241, f="PracticeRobotParameters") -> (s? t:f=w122:T2)
    n92 = global read "Global_Var_Other.vi" "Auto_Enable_Manual?"() -> (w214:bool)
    n93 = Or(x=w158, y=w214) -> (x .or. y?=w215:bool)
    n94 = Unbundle By Name(w334) -> ("Joystick_1.Joystick_F/B"=w254:dbl, "Joystick_1.Joystick_L/R_Turn"=w190:dbl, "Joystick_1.Joystick_Intake"=w338:bool, "Joystick_2.Joystick_Intake_B"=w343:bool)
    n95 = global read "Global_Var_Other.vi" "Auto_Enable?"() -> (w154:bool)
    n96 = global write "Global_Var_Other.vi" "Auto_Enable?"(w215) -> ()
    n97 = Or(x=w222, y=w223) -> (x .or. y?=w224:bool)
    n98 = global write "GlobalVar_LED.vi" "Win"(w209) -> ()
    n99 = Or(x=w337, y=w154) -> (x .or. y?=w152:bool)
    n100 = Unbundle By Name(w122) -> ("Invert_Intake"=w238:bool)
    n101 = call "Debounce.vi"("Input"=w179, "Num samples"=5) -> ("Output"=w175:bool)  [unwired: 1 in]
    n102 = call "Joystick.vi"() -> ("Joysticks"=w310:T48)  [unwired: 1 in]
    n103 = call "Shifters.vi"("High Gear"=w152, "ShifterDevRef"=w314) -> ()  [unwired: 1 in]
    n104 = Or(x=w312, y=w335) -> (x .or. y?=w251:bool)
    n105 = Or(x=w335, y=w336) -> ()  [unwired: 1 out]
    n106 = Or(x=w311, y=w312) -> (x .or. y?=w170:bool)
    n107 = Unbundle By Name(w157) -> ("Sensors.IMU.ADI IMU Interrupt DevRef"=w350:T21)
    n108 = call "PixyCam_Get_Targets.vi"("PixyCamDevRef"=w308) -> ()  [unwired: 4 in, 3 out]
    n109 = global read "Global_Var_Other.vi" "Drive_PID_Enable?"() -> (w150:bool)
    n110 = global read "Global_Var_Other.vi" "Drive_Speed_Auto"() -> (w181:dbl)
    n111 = call "Intake_Motor.vi"("Forward_Button_Pushed?"=w338, "Reverse_Button_Pushed?"=w343, "Invert?"=w238, "MotorControlDevRef"=w324, "Intake_Motor_Limit_Forward"=1.0, "Intake_Motor_Limit_Backward"=-1.0) -> ()  [unwired: 10 in]
    n112 = call <vilib>:"WPI_DigitalInputGetValue.vi"("DigitalInputDevRef"=w264) -> ("Value"=w262:bool)  [unwired: 8 in, 2 out]
    n113 = Unbundle By Name(w310) -> ("Joystick_2.Joystick_Turret_L/R"=w309:dbl)
    n114 = global write "GlobalVar_LED.vi" "Climbing"(w208) -> ()
    n115 = call "ADI_IMU_ADIS16448_Get Angles.vi"("ADI IMU Interrupt DevRef"=w350) -> ("IMU Angles Out"=w349:T10)  [unwired: 7 in, 3 out]
    "IMU Angles Out" <- w349
    n116 = Unbundle By Name(w349) -> ("Z Angle"=w346:dbl)
    n117 = global read "Global_Var_Other.vi" "Auto_Enable?"() -> (w169:bool)
    n118 = call "Climber_Motor.vi"("Invert?"=FALSE, "Climb_Up?"=w208, "MotorControlDevRef"=w318) -> ()  [unwired: 9 in]
    n119 = global read "Global_Var_Other.vi" "ShooterSpeed_Auto"() -> (w171:dbl)
    n120 = call "Debounce.vi"("Input"=w262, "Num samples"=10) -> ()  [unwired: 1 in, 1 out]
    n121 = call "Debounce.vi"("Input"=w150, "Num samples"=10) -> ()  [unwired: 1 in, 1 out]
    n122 = Unbundle By Name(w122) -> ("Feeder_Invert"=w236:bool)
    n123 = call "dashboardNames.vi"() -> ("String Names"=w118:string[])  [unwired: 8 in, 3 out]
    n124 = global read "Global_Var_Other.vi" "RunFeeder_Auto"() -> (w168:bool)
    n125 = Unbundle By Name(w122) -> ("Drive PID Gains"=w105:T45, "DriveSpeed_Invert"=w237:bool)
    n126 = feedback #1() -> (w347:dbl)  [unwired: 1 in]
    n127 = Select(t=w347, s=w150, f=w346) -> (s? t:f=w305:dbl)
    n128 = feedback-in #1(w305) -> ()
    n129 = Not(x=w251) -> (.not. x?=w252:bool)
    n130 = And(x="Gear_Beam_Break_Sensor_Triggered", y=w224) -> (x .and. y?=w261:bool)
    n131 = call "dashboardNames.vi"() -> ("String Names"=w127:string[], "Slider Names"=w147:string[])  [unwired: 8 in, 2 out]
    n132 = Select(t=w171, s=w169, f=0.0) -> (s? t:f=w172:dbl)
    n133 = Unbundle(w105) -> ("proportional gain (Kc)"=w111:dbl, "integral time (Ti, min)"=w110:dbl, "derivative time (Td, min)"=w109:dbl)
    n134 = Unbundle By Name(w122) -> ("DefaultDBParams.RedAllianceRPM"=w121:dbl, "DefaultDBParams.BlueAllianceRPM"=w120:dbl, "DefaultDBParams.BaselineRPM"=w103:dbl)
    n135 = Select(t=w252, s=w236, f=w251) -> (s? t:f=w230:bool)
    n136 = Greater Or Equal?(x=w309, y=0.6) -> (x >= y?=w342:bool)
    n137 = Less Or Equal?(x=w309, y=-0.6) -> (x <= y?=w341:bool)
    n138 = global read "Global_Var_Other.vi" "Auto_Enable?"() -> (w180:bool)
    n139 = Select(t=w181, s=w180, f=w254) -> (s? t:f=w182:dbl)
    n140 = Negate(x=w182) -> (-x=w253:dbl)
    n141 = global read "Global_Var_Other.vi" "Turn_Speed_Auto"() -> (w184:dbl)
    n142 = call "Shooter_Motor.vi"("LeftMotorControlDevRef"=w317, "RightMotorControlDevRef"=w228, "ShooterSpeed"=w172, "Shooter_Forward?"=w193) -> ()  [unwired: 16 in]
    n143 = call "time_delta.vi"() -> ("dt (s)"=w245:dbl)  [unwired: 1 in]
    n144 = Index Array(array=w118, index #1=dbStringDisplayNames_Type."Drive P" ("DBSliderDispNames"), index #2=dbStringDisplayNames_Type."Drive I" ("DBSliderDispNames"), index #3=dbStringDisplayNames_Type."Drive D" ("DBSliderDispNames")) -> (element #1=w114:string, element #2=w113:string, element #3=w112:string)
    n145 = Select(t=w253, s=w237, f=w182) -> (s? t:f=w220:dbl)
    n146 = Select(t=w168, s=w169, f=w170) -> (s? t:f=w160:bool)
    n147 = call "Joystick.vi"() -> ("Joysticks"=w319:T48)  [unwired: 1 in]
    n148 = global read "Global_Var_Other.vi" "Auto_Enable?"() -> (w217:bool)
    n149 = call "DBReadStringAsNumber.vi"("DBControlName"=w114, "Default Value"=w111) -> ("Value"=w108:dbl)
    n150 = call "DBReadStringAsNumber.vi"("DBControlName"=w113, "Default Value"=w110) -> ("Value"=w107:dbl)
    n151 = call "DBReadStringAsNumber.vi"("DBControlName"=w112, "Default Value"=w109) -> ("Value"=w106:dbl)
    n152 = call "Shooter_Turret_Motor.vi"("MotorControlDevRef"=w313, "Turret_Clockwise?"=w342, "Turret_Counterclockwise?"=w341) -> ("TurretPosReached"=w196:bool)  [unwired: 23 in, 1 out]
    n153 = global write "GlobalVar_LED.vi" "Shooting"(w160) -> ()
    n154 = call "Feeder_Motor.vi"("Shooter_Feeder_Motor_Limit"=1.0, "Feeder_Button_Pressed?"=w160, "Invert?"=w230, "BottomMotorDevRef"=w316) -> ()  [unwired: 2 in, 1 out]
    n155 = Select(t=w184, s=w180, f=w190) -> (s? t:f=w191:dbl)
    n156 = Index Array(array=w147, index #1=dbSliderDisplayNames_Type."AutoSpeed" ("DBSliderDispNames"), index #2=dbSliderDisplayNames_Type."MiddleAutoDist (in)" ("DBSliderDispNames"), index #3=dbSliderDisplayNames_Type."SideAutoDist (in)" ("DBSliderDispNames")) -> (element #1=w144:string, element #2=w143:string, element #3=w140:string)
    n157 = Index Array(array=w127, index #1=dbStringDisplayNames_Type."RedAllianceRPM" ("DBSliderDispNames"), index #2=dbStringDisplayNames_Type."BlueAllianceRPM" ("DBSliderDispNames"), index #3=dbStringDisplayNames_Type."BaselineRPM" ("DBSliderDispNames")) -> (element #1=w124:string, element #2=w123:string, element #3=w101:string)
    n158 = Not(x=w152) -> (.not. x?=w151:bool)
    n159 = Bundle(cluster=w105, "proportional gain (Kc)"=w108, "integral time (Ti, min)"=w107, "derivative time (Td, min)"=w106) -> (w104:T45)
    n160 = global read "Global_Var_Other.vi" "Gear_Rail_Pos_Reached?"() -> (w288:bool)
    n161 = global read "Global_Var_Other.vi" "Shooter_RPM_Reached?"() -> (w328:bool)
    n162 = Unbundle By Name(w319) -> ("Joystick_1.Joystick_Place_Gear"=w213:bool, "Joystick_1.Joystick_Aim"=w330:bool, "Joystick_1.Joysick_Shoot"=w327:bool)
    n163 = global read "Global_Var_Other.vi" "Place_Gear_Auto?"() -> (w212:bool)
    n164 = global read "Global_Var_Other.vi" "Turret_Pos_Reached?"() -> (w329:bool)
    n165 = global write "Global_Var_Other.vi" "Turret_Pos_Reached?"(w196) -> ()
    n166 = global write "GlobalVar_LED.vi" "TurretAimed"(w196) -> ()
    n167 = call "Argo_Drive.vi"("Speed_Main"=w220, "Turning_PID_Enable"=w150, "PID Gains"=w104, "Turning_Main"=w191, "Auto_Enable"=w217, "High_Gear"=w151, "Quick_Turn"=TRUE, "Turning_Setpoint"=w305, "dt (s)"=w245, "Yaw"=w346) -> ("Left_Motor"=w355:dbl, "Right_Motor"=w354:dbl)  [unwired: 8 in]
    n168 = Unbundle By Name(w157) -> ("Motors.Drive_Motor.RobotDriveDevRef"=w356:T11)
    n169 = call "ADI_IMU_ADIS16448_Get Angles.vi"("ADI IMU Interrupt DevRef"=w257) -> ("IMU Angles Out"=w256:T10)  [unwired: 7 in, 3 out]
    n170 = call "dashboardNames.vi"() -> ("Slider Names"=w139:string[])  [unwired: 8 in, 3 out]
    n171 = Index Array(array=w139, index=dbSliderDisplayNames_Type."RailCenterOffset (in)" ("DBSliderDispNames")) -> (element=w137:string)
    n172 = Unbundle By Name(w256) -> ("Z Angle"=w255:dbl)
    n173 = Or(x=w212, y=w213) -> (x .or. y?=w211:bool)
    n174 = call-poly <vilib>:"NT Read Value.vi"("Default Value"="Reverse_Drive_Speed", "Name"=w144) -> ("Numeric"=w132:dbl)  [unwired: 8 in, 1 out]
    n175 = call-poly <vilib>:"NT Read Value.vi"("Default Value"="Reverse_Drive_Distance", "Name"=w143) -> ("Numeric"=w131:dbl)  [unwired: 8 in, 1 out]
    n176 = call-poly <vilib>:"NT Read Value.vi"("Default Value"="Continue_Forward_Distance", "Name"=w140) -> ("Numeric"=w130:dbl)  [unwired: 8 in, 1 out]
    n177 = call "DBReadStringAsNumber.vi"("DBControlName"=w124, "Default Value"=w121) -> ("Value"=w129:dbl)
    n178 = call "DBReadStringAsNumber.vi"("DBControlName"=w123, "Default Value"=w120) -> ("Value"=w128:dbl)
    n179 = call "DBReadStringAsNumber.vi"("DBControlName"=w101, "Default Value"=w103) -> ("Value"=w100:dbl)
    n180 = call-poly <vilib>:"NT Read Value.vi"("Default Value"=0.0, "Name"=w137) -> ("Numeric"=w135:dbl)  [unwired: 8 in, 1 out]
    n181 = global read "Global_Var_Other.vi" "Gear_Gate_Pos_Reached?"() -> (w332:bool)
    n182 = global read "Global_Var_Other.vi" "Gear_Rail_Pos_Reached?"() -> (w333:bool)
    n183 = global read "Global_Var_Other.vi" "Gear_Pusher_Finished?"() -> (w331:bool)
    n184 = feedback #2() -> (w166:bool)  [unwired: 1 in]
    n185 = And(x=w166, y="StartGearCollect") -> (x .and. y?=w276:bool)
    n186 = call "Shooter_Operator_Assist.vi"("Turret Aimed"=w329, "Shooter Motor Speed Good"=w328, "Shoot Command"=w327, "Start"=TRUE) -> ()  [unwired: 8 in, 4 out]
    n187 = call "TurretAim_OperatorAssist.vi"("Reacquire"=w330, "Start"=TRUE) -> ("Current_State"=w192:T49)  [unwired: 5 in, 1 out]
    n188 = Or(x="ResetGearPlacer", y=w175) -> (x .or. y?=w177:bool)
    n189 = global write "GlobalVar_LED.vi" "Turret_State"(w192) -> ()
    n190 = global read "Global_Var_Other.vi" "Encoder_Dist_Travelled"() -> (w259:dbl)
    n191 = Unbundle By Name(w122) -> ("Rail Parameters.CatchPosition"=w159:dbl)
    n192 = call "GearCollecter_OperatorAssist.vi"("CatchPosition"=w159, "ReturnToCatch"=w175, "CarriageReturned"=w288, "Manual_Overide"="ResetGearCollect", "Start"=w276, "Gear_Beam_Break_Sensor_Triggered"=w261) -> ("Gear_Rail_Position"=w286:dbl, "GearChuteExtend"=w298:bool, "Catch_Complete?"=w258:bool, "Gate_Pos"=w284:T9, "Current_State"=w194:T41)  [unwired: 1 in]
    n193 = global write "GlobalVar_LED.vi" "GearCatch_State"(w194) -> ()
    n194 = global read "Global_Var_Other.vi" "YoYo_Value"() -> (w248:dbl)
    n195 = call "RobotDriveMotors.vi"("RightSpeed"=w354, "LeftSpeed"=w355, "RobotDriveDevRef"=w356) -> ()  [unwired: 6 in, 3 out]
    n196 = Bundle By Name(cluster=T7 {"MiddleAutoDist (in)"=0.0, "SideAutoDist (in)"=0.0, "AutoSpeed"=0.0, "RailCenterOffset (in)"=0.0, "RedAllianceRPM"=0.0, "BlueAllianceRPM"=0.0, "BaselineRPM"=0.0} ("DBParams"), "AutoSpeed"=w132, "MiddleAutoDist (in)"=w131, "SideAutoDist (in)"=w130, "RedAllianceRPM"=w129, "BlueAllianceRPM"=w128, "BaselineRPM"=w100) -> (w133:T7)
    n197 = call-poly <vilib>:"NT Read Value.vi"("Name"="Auto Selector") -> ("String"=w187:string)  [unwired: 9 in, 1 out]
    n198 = global read "Global_Var_Other.vi" "Auto_Enable?"() -> (w216:bool)
    n199 = And(x="StartGearPlace", y=w258) -> (x .and. y?=w278:bool)
    n200 = Select(t="GearRailWantedPosition", s="Manual_Track_Position", f=w248) -> (s? t:f=w249:dbl)
    n201 = call <vilib>:"WPI_DriverStationGet Alliance Info.vi"() -> ("Alliance"=w119:T50)  [unwired: 10 in, 1 out]
    n202 = Scan From String(input string=w187, default 1="AutoMode") -> (output 1=w183:T1)  [unwired: 3 in, 3 out]
    n203 = global write "GlobalVar_LED.vi" "AutoMode"(w183) -> ()
    n204 = Unbundle By Name(w157) -> ("Sensors.Pots.Gear_Gate_Pot.AIDeviceRef"=w301:T25)
    n205 = Unbundle By Name(w157) -> ("Sensors.Pots.Gear_Rail_Pot.AIDeviceRef"=w344:T25)
    n206 = Unbundle By Name(w157) -> ("Sensors.DIOs.Gear_Orientation_Beambreak.DigitalInputDevRef"=w268:T33, "Motors.Gear_Rail_Motor.MotorControlDevRef"=w323:T12, "Pneumatics.Gear_Chute.SolenoidDevRef"=w322:T36, "Motors.Gear_Gate_Motor.MotorControlDevRef"=w321:T12, "Sensors.Ultrasonics.Gear_Peg_Ultrasonic.SonarMB1010DigitalDevRef"=w244:T27)
    n207 = Unbundle By Name(w319) -> ("Joystick_2.Joystick_GearChute"=w231:bool, "Joystick_2.Joystick_GateOpen"=w304:bool, "Joystick_2.Joystick_GateClose"=w303:bool)
    n208 = Not(x=w258) -> (.not. x?=w272:bool)
    n209 = Or(x=w231, y="Manual") -> (x .or. y?=w233:bool)
    n210 = And(x="Collect", y=w272) -> (x .and. y?=w273:bool)
    n211 = call "PotRead.vi"("PotDevRef"=w301) -> ("Pot"=w300:dbl)  [unwired: 4 in, 1 out]
    n212 = Or(x=w231, y=w293) -> (x .or. y?=w299:bool)
    n213 = Unbundle By Name(w122) -> ("GateParameters"=w234:T3)
    n214 = global write "Global_Var_Other.vi" "Auto_Enable_Manual?"("Start_Auto?") -> ()
    n215 = call "YoYoRead.vi"("YoYoDevRef"=w344) -> ("YoYo"=w307:dbl, "In_Range?"=w306:bool)  [unwired: 1 in]
    n216 = global read "Global_Var_Other.vi" "YoYo_Value"() -> (w200:dbl)
    n217 = Unbundle By Name(w122) -> ("Rail Parameters.Scale Positions.Forward_Limit"=w205:dbl, "Rail Parameters.Scale Positions.Reverse_Limit"=w204:dbl)
    n218 = Unbundle By Name(w122) -> ("Rail Parameters"=w235:T5)
    n219 = Unbundle By Name(w122) -> ("UltrasonicParameters"=w207:T6)
    n220 = Unbundle By Name(w122) -> ("Rail Parameters.Scale Positions.Forward_Limit"=w199:dbl, "Rail Parameters.Scale Positions.Reverse_Limit"=w198:dbl)
    n221 = call <vilib>:"WPI_DigitalInputGetValue.vi"("DigitalInputDevRef"=w268) -> ("Value"=w267:bool)  [unwired: 8 in, 2 out]
    n222 = call "time_delta.vi"() -> ("dt (s)"=w201:dbl)  [unwired: 1 in]
    n223 = global read "Global_Var_Other.vi" "Auto_Enable?"() -> (w153:bool)
    n224 = global write "Global_Var_Other.vi" "YoYo_Value"(w307) -> ()
    n225 = global write "Global_Var_Other.vi" "YoYo_In_Range?"(w306) -> ()
    n226 = call "Debounce.vi"("Input"=w267, "Num samples"=10) -> ("Output"=w265:bool)  [unwired: 1 in]
    "Gear_Orientation_Bb_True?" <- w265
    n227 = global write "Global_Var_Other.vi" "Gear_Orientation_Bb_True?"(w265) -> ()
    n228 = call "UltraRead.vi"("UltrasonicParameters"=w207, "SonarMB1010DigitalDevRef"=w244) -> ("Unfiltered_UltrasonicRange (in)"=w242:dbl, "MedianOnly_UltrasonicRange (in)"=w243:dbl, "UltrasonicRange (in)"=w206:dbl)  [unwired: 3 in]
    "Distance" <- w206
    n229 = call "Gear_Placer_OperatorAssist.vi"("Start?"=w278, "Reset?"=w177, "Ultrasonic"=w206, "Rail_Finished?"=w333, "Gate_Finished?"=w332, "Gear_Pusher_Finished?"=w331, "Place_Gear?"=w211, "RailTargetClamp"=w159, "GearMiddleOffset"=w135) -> ("Returning"=w167:bool, "Place_Complete?"=w210:bool, "Rail_Target_Position"=w285:dbl, "Gate_Pos"=w281:T9, "Gear_Pusher_Extend?"=w291:bool, "Gear_Chute_Extend?"=w294:bool, "State"=w195:T51)  [unwired: 2 in, 2 out]
    n230 = feedback-in #2(w210) -> ()
    n231 = Build Array(w249, w286, w285) -> (w287:dbl[])
    n232 = Build Array(w293, FALSE, w291) -> (w292:bool[])
    n233 = global write "GlobalVar_LED.vi" "GearPlace_State"(w195) -> ()
    n234 = call "Place_Middle_Gear_Auto.vi"("Encoder_In"=w259, "Yaw_In"=w255, "DBParams"=w133, "Place_Finished?"=w167, "Alliance"=w119, "Turning_Angle"="Turning_Angle", "Start?"=w216, "AutoMode"=w183) -> ("ShooterSpeedOutput (rpm)"=w174:dbl, "RunFeeder"=w173:bool, "Turning_Speed"=w189:dbl, "Drive_PID_Enable"=w221:bool, "Place_Gear?"=w226:bool, "Drive_Speed"=w227:dbl)  [unwired: 4 in, 2 out]
    n235 = Build Array("Manual_Gate_Control", w284, w281) -> (w283:T9[])
    n236 = Not(x=w210) -> (.not. x?=w269:bool)
    n237 = And(x="Place", y=w269) -> (x .and. y?=w270:bool)
    n238 = global write "Global_Var_Other.vi" "Drive_PID_Enable?"(w221) -> ()
    n239 = global write "Global_Var_Other.vi" "Place_Gear_Auto?"(w226) -> ()
    n240 = global write "Global_Var_Other.vi" "Drive_Speed_Auto"(w227) -> ()
    n241 = global write "Global_Var_Other.vi" "Turn_Speed_Auto"(w189) -> ()
    n242 = global write "Global_Var_Other.vi" "RunFeeder_Auto"(w173) -> ()
    n243 = global write "Global_Var_Other.vi" "ShooterSpeed_Auto"(w174) -> ()
    n244 = Build Array(w299, w298, w294) -> (w297:bool[])
    n245 = Build Array(w233, w273, w270) -> (w279:bool[])
    n246 = call-poly "Arbitor.vi"("Selector Array"=w279, "Input Array"=w287) -> ("Arbitrated Output"=w202:dbl)
    n247 = call-poly "Arbitor.vi"("Selector Array"=w279, "Input Array"=w292) -> ("Arbitrated Output"=w289:bool)
    n248 = call "Gear pusher.vi"("Extend"=w289, "Cylinder_Devref"=w315) -> ()  [unwired: 3 in]
    n249 = call-poly "Arbitor.vi"("Selector Array"=w279, "Input Array"=w283) -> ("Arbitrated Output"=w282:i32)
    n250 = call-poly "Arbitor.vi"("Selector Array"=w279, "Input Array"=w297) -> ("Arbitrated Output"=w296:bool)
    n251 = call "Gear_Chute.vi"("SolenoidDevRef"=w322, "Extend?"=w296) -> ()  [unwired: 10 in]
    n252 = call "Gear_Gate.vi"("MotorControlDevRef"=w321, "Open_Button_Pressed?"=w304, "GateParameters"=w234, "Close_Button_Pressed?"=w303, "Potentiometer_Input"=w300, "Gate_Pos"=w282) -> ("Reached"=w302:bool)  [unwired: 21 in]
    "GateReached" <- w302
    n253 = call "Gear_Rail.vi"("MotorControlDevRef"=w323, "dt_In_PID"=w201, "Potentiometer_Input"=w200, "Potentiometer_WantedPos"=w202, "Rail Parameters"=w235) -> ()  [unwired: 22 in, 1 out]
    n254 = global write "Global_Var_Other.vi" "Gear_Gate_Pos_Reached?"(w302) -> ()
    n255 = case shown="True" w153 {
      selector: w153 -> [_ w359]
      frame False {
      }
      frame True {
        n256 = global write "Global_Var_Drive.vi" "Joystick_MiddleRailAllign"(w359) -> ()
        n257 = global write "Global_Var_Other.vi" "Rail_To_Middle"(w359) -> ()
      }
    }
    n258 = Bundle("UltrasonicRange (in)"=w206, "MedianOnly_UltrasonicRange (in)"=w243, "Unfiltered_UltrasonicRange (in)"=w242) -> (→"Ultrasonic":T8)  [unwired: 1 in]
    n259 = call "NumToPercent.vi"("MaxVal"=w205, "MaxOut"=u8 99, "MinVal"=w204, "CurVal"=w202, "MinOut"=u8 0) -> ("IntPercent"=w203:u8)
    n260 = global write "GlobalVar_LED.vi" "UltraPosition"(w203) -> ()
    n261 = call "NumToPercent.vi"("MaxVal"=w199, "MaxOut"=u8 99, "MinVal"=w198, "CurVal"=w200, "MinOut"=u8 0) -> ("IntPercent"=w197:u8)
    n262 = global write "GlobalVar_LED.vi" "YoYoPosition"(w197) -> ()
    n263 = Wait (ms)(milliseconds to wait=u32 40) -> ()  [unwired: 1 out]
  }
  n264 = Unbundle By Name(w2) -> ("Sensors.PixyCam.PixyCamDevRef Out"=w1:T16)
  n265 = call "PixyCam_Loop.vi"("PixyCamDevRef"=w1) -> ()  [unwired: 5 in, 2 out]
